vi "VIH Platform - LabVIEW - Library - Get License Status.vi"(8 "error in":errorcluster, 11 "Library Refnum":refnum<vi>) -> (0 "error out":errorcluster, 2 "License Status":u32(ring) items=["Failure", "Activated Success", "Demo Success", "Full Demo Success"], 3 "dup Library Refnum":refnum<vi>)   [LabVIEW 2014]
doc: "::: VI Helpeks :::\nCopyright (c) 2000-2026 Konstantin Shifershteyn. All rights reserved."
panel:
  # "VI Helpeks\nCopyright (c) 2012-2026 Konstantin Shifershteyn"
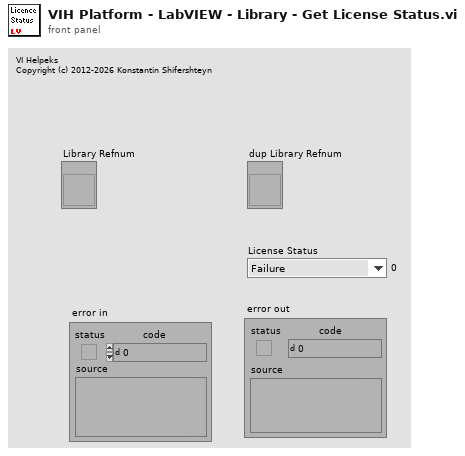
[diagram p1: front panel]
types:
  T1 = enum32{"Failure", "Activated Success", "Demo Success", "Full Demo Success"}
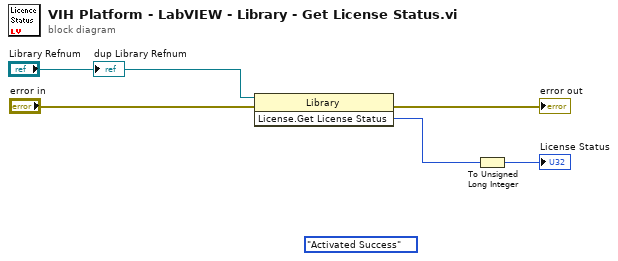
[diagram p0: block diagram]
diagram:
  (unwired) T1."Activated Success" ("License:Get License Status")
  n1 = invoke class="Library" method="License.Get License Status"(reference="Library Refnum", error in="error in") -> (error out=→"error out":errorcluster, "License.Get License Status"=w1:T1)  [unwired: 1 in, 1 out]
  n2 = To Unsigned Long Integer(number=w1) -> (unsigned 32bit integer=→"License Status":u32)
  "dup Library Refnum" <- "Library Refnum"
